vi "Initialize.vi"(8 "error in (no error)":errorcluster, 11 "UserEventActivationHandler in":refnum<class "UserEventActivationHandler.lvclass">) -> (0 "error out":errorcluster, 3 "UserEventActivationHandler out":refnum<class "UserEventActivationHandler.lvclass">)   [LabVIEW 2026, in "ToastNotification.lvlib" / "UserEventActivationHandler.lvclass"]
doc: "Create the typed User Event used to relay activation data to the calling application, and store its reference in this handler. The payload contains Activation and its conversion error. Called by ToastService.Initialize; retrieve Event Ref from the returned initialized handler. Skips creation on incoming error. The current implementation does not guard against repeated initialization; initialize once per owned handler lifecycle."
uses:
  UserEventActivationHandler.lvclass
  Activation Event Data.ctl
  ToastNotification/Activation.ctl
  ToastNotification/Argument.ctl
  UserEventActivationHandler.lvclass/UserEventActivationHandler.ctl
  Write Event Ref.vi
  ToastNotification/ToastNotification.lvlib
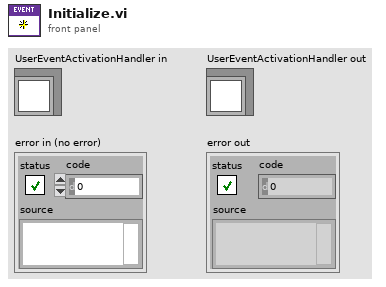
[diagram p1: front panel]
types:
  T1 = typedef "ToastNotification.lvlib/UserEventActivationHandler.lvclass/Activation Event Data.ctl" = cluster{"Activation":T2, "error":errorcluster}
  T2 = typedef "ToastNotification.lvlib/Activation.ctl" = cluster{"Arguments":string, "User Inputs":T3[]}
  T3 = typedef "ToastNotification.lvlib/Argument.ctl" = cluster{"Key":string, "Value":string}
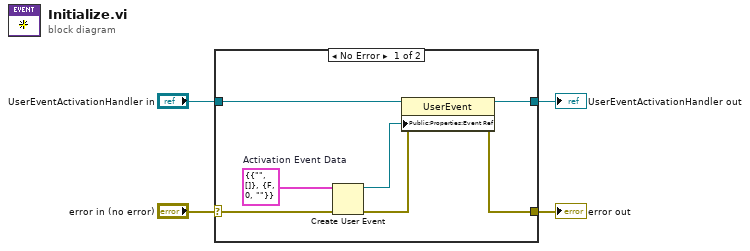
[diagram p0: block diagram]
diagram:
  n1 = case shown="No Error" "error in (no error)" {
    selector: "error in (no error)" -> [w10 w13]
    tunnel: [w9 w12] -> w3
    tunnel: "UserEventActivationHandler in" -> [w11 w12]
    tunnel: [w7 w13] -> w1
    frame No Error {
      w5 = T1 {"Activation"={"Arguments"="", "User Inputs"=[]}, "error"={"status"=FALSE, "code"=0, "source"=""}}  # Activation Event Data
      n2 = Create User Event(user event datatype=w5, error in=w10) -> (user event=w6:refnum<user-event>, error out=w8:errorcluster)
      n3 = property class="UserEvent"(reference=w11, error in=w8, "Public:Properties:Event Ref"=w6) -> (reference out=w9:refnum<class "UserEventActivationHandler.lvclass">, error out=w7:errorcluster)
    }
    frame Error {
    }
  }
  "error out" <- w1
  "UserEventActivationHandler out" <- w3
